vi "suhas&claire-mainencoder.vi"() -> ()   [LabVIEW 2026]
uses:
  <vilib>/DAQmx/read.llb/DAQmx Read (Counter DBL 1Chan 1Samp).vi
  <vilib>/Utility/file.llb/Write Delimited Spreadsheet (string).vi
  <vilib>/DAQmx/miscellaneous.llb/DAQmx Fill In Error Info.vi
panel:
  out "Invert X":bool
  in  "Motor Clock Num per Pulse":u32=100
  in  "Port0 Bits 2":tag="Dev1/port0/line0:7"
  in  "Laser Sync Source":tag="/Dev1/PFI8"
  in  "Laser DO Rate":u32=40000
  in  "Motor Pulse Rate 2":i32=200
  in  "kx":dbl=1.0
  in  "Move X 2":bool
  in  "delta_x 2":dbl=1.0
  in  "xdir 2":bool=TRUE
  out "Y Velocity (mm/s)":dbl
  out "Y Position (mm)":dbl
  out "Time Between Pulse":dbl
  in  "stop":bool
  out "Logging":bool
  out "Saving to":path
  out "XY Graph":cluster{i16[], dbl[]}(graph)
  out "Pulse Count":dbl
  out "X Velocity (mm/s)":dbl
  out "X Position (mm)":dbl
  # "mm"
  # "mm/s"
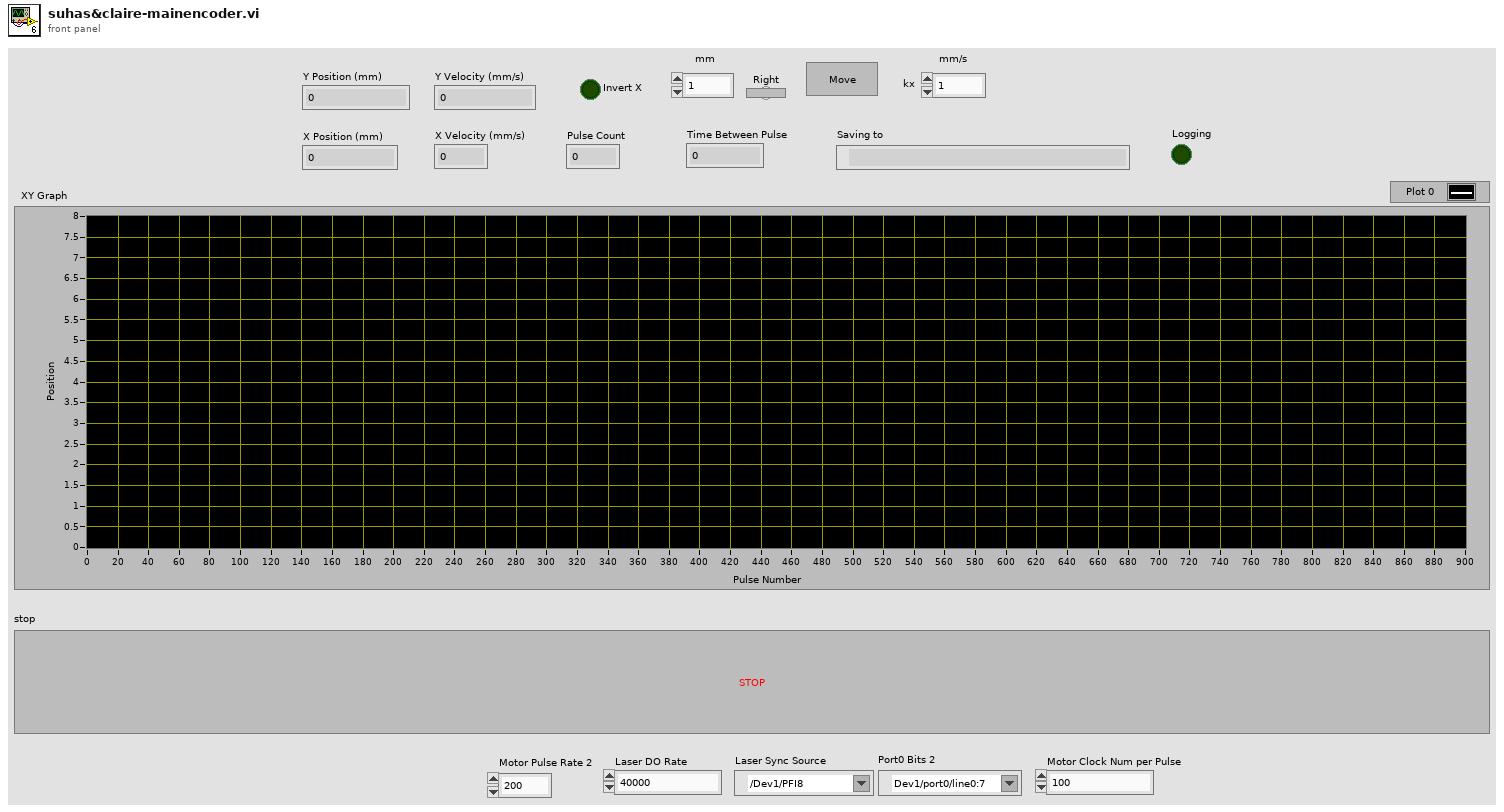
[diagram p1: front panel]
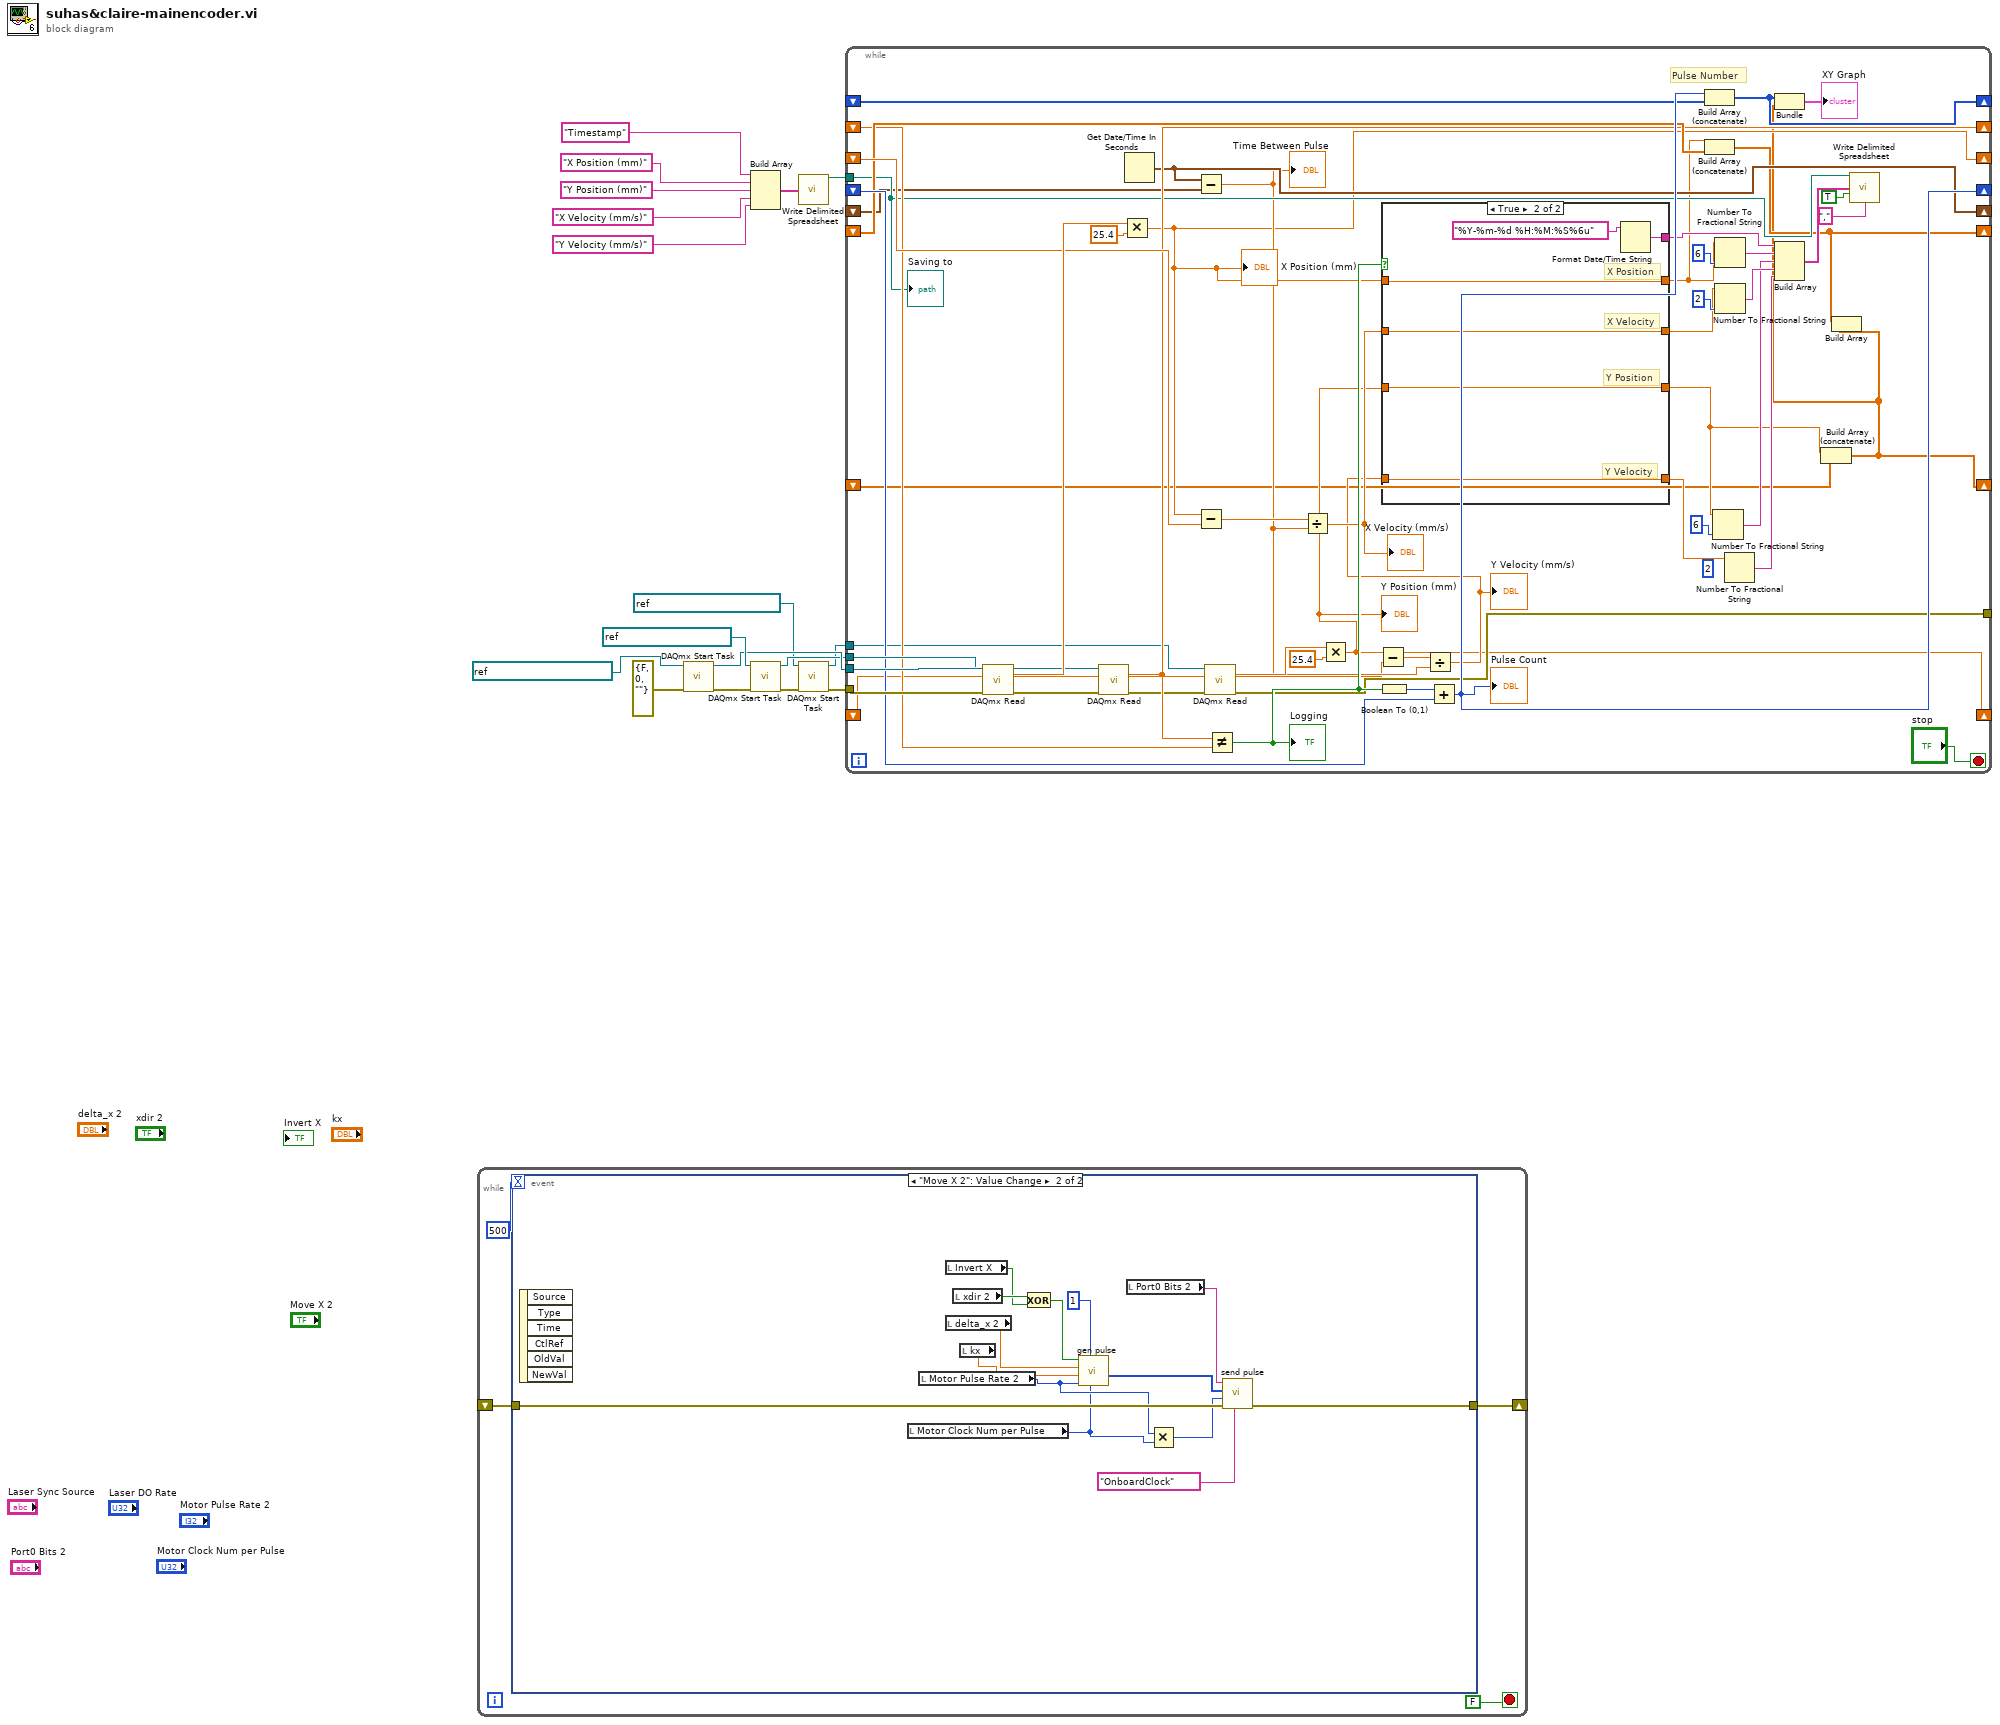
[diagram p0: block diagram]
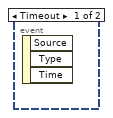
[diagram p2: hidden frame]
diagram:
  n1 = while {
    shift-right: [w20] -> _
    shift-left: _ -> [w19]
    stop <- FALSE stop-if-true
    n2 = event shown="[1] \"Move X 2\": Value Change" {
      selector: _ -> [_ _]
      dyn-events: _ -> [_ _]
      timeout: 500 -> [_ _]
      tunnel: [_ w35] -> w20
      tunnel: w19 -> [_ w34]
      event Timeout {
        n3 = event-data() -> ()  [unwired: 1 in, 3 out]
      }
      event "Move X 2": Value Change {
        n4 = event-data() -> ()  [unwired: 1 in, 6 out]
        n5 = local read "Motor Clock Num per Pulse"() -> (w27:u32)
        n6 = local read "Motor Pulse Rate 2"() -> (w28:i32)
        n7 = local read "Invert X"() -> (w22:bool)
        n8 = local read "delta_x 2"() -> (w32:dbl)
        n9 = local read "xdir 2"() -> (w24:bool)
        n10 = local read "kx"() -> (w31:dbl)
        n11 = Exclusive Or(1:w22, 2:w24) -> (0:w23:bool)
        n12 = call "gen pulse.vi"("clk per pulse"=w27, "bit"=u8 1, "Motor Pulse Rate / mm"=w28, "kx"=w31, "xn"=w32, "dir"=w23) -> ("pulsetrain"=w30:u8[])  [unwired: 3 in, 2 out]
        n13 = local read "Port0 Bits 2"() -> (w29:tag)
        n14 = Multiply(x=w28, y=w27) -> (x*y=w26:u32)
        n15 = call "send pulse.vi"("source"=tag "OnboardClock", "error in"=w34, "Motors DO rate"=w26, "P0 DO data"=w30, "Port0 Bits"=w29) -> ("error out"=w35:errorcluster)  [unwired: 6 in]
      }
    }
  }
  n16 = call <vilib>:"DAQmx Start Task.vi"("task/channels in"=refnum<k21> "MyLinearPositionTask", "error in"=errorcluster {"status"=FALSE, "code"=0, "source"=""}) -> ("task out"=w14:refnum<k21>, "error out"=w8:errorcluster)  [unwired: 12 in]
  n17 = Build Array("Timestamp", "X Position (mm)", "Y Position (mm)", "X Velocity (mm/s)", "Y Velocity (mm/s)") -> (w10:string[])
  n18 = call <vilib>:"DAQmx Start Task.vi"("task/channels in"=refnum<k21> "MyCountEdgesTask", "error in"=w8) -> ("task out"=w13:refnum<k21>, "error out"=w3:errorcluster)  [unwired: 12 in]
  n19 = call-poly <vilib>:"Write Delimited Spreadsheet.vi"("1D data"=w10) -> ("new file path (Not A Path if cancelled)"=w9:path)  [unwired: 13 in, 1 out]
  n20 = call <vilib>:"DAQmx Start Task.vi"("task/channels in"=refnum<k21> "MyLinearPositionTaskY", "error in"=w3) -> ("task out"=w1:refnum<k21>, "error out"=w2:errorcluster)  [unwired: 12 in]
  n21 = while {
    tunnel: w2 -> [w86]
    tunnel: w14 -> [w85]
    tunnel: w13 -> [w82]
    shift-right: [w72] -> _
    shift-left: _ -> [w71]
    shift-right: [w48] -> _
    shift-left: _ -> [w80]
    shift-right: [w76] -> _
    shift-left: _ -> [w77]
    shift-right: [w70] -> _
    shift-left: _ -> [w75]
    shift-right: [w37] -> _
    shift-left: _ -> [w74]
    tunnel: w9 -> [w62]
    shift-right: [w61] -> _
    shift-left: _ -> [w60]
    tunnel: w1 -> [w59]
    tunnel: [w57] -> _
    shift-right: [w43] -> _
    shift-left: _ -> [w42]
    shift-right: [w36] -> _
    shift-left: _ -> [w38]
    stop <- "stop" stop-if-true
    (unwired) i16 2 ("precision (6)")
    # "Pulse Number"
    n22 = call-poly <vilib>:"DAQmx Read.vi"("task/channels in"=w85, "error in"=w86) -> ("data"=w84:dbl, "error out"=w81:errorcluster)  [unwired: 11 in, 1 out]
    n23 = call-poly <vilib>:"DAQmx Read.vi"("task/channels in"=w82, "error in"=w81) -> ("data"=w72:dbl, "error out"=w58:errorcluster)  [unwired: 11 in, 1 out]
    n24 = Multiply(x=w84, y=25.4) -> (x*y=w48:dbl)
    "X Position (mm)" <- w48
    n25 = Get Date/Time In Seconds() -> (seconds since 1Jan1904=w61:timestamp)
    n26 = Subtract(x=w61, y=w60) -> (x-y=w53:dbl)
    "Time Between Pulse" <- w53
    n27 = Subtract(x=w48, y=w80) -> (x-y=w79:dbl)
    n28 = call-poly <vilib>:"DAQmx Read.vi"("task/channels in"=w59, "error in"=w58) -> ("data"=w56:dbl, "error out"=w57:errorcluster)  [unwired: 11 in, 1 out]
    n29 = Not Equal?(x=w72, y=w71) -> (x != y?=w73:bool)
    "Logging" <- w73
    n30 = Divide(x=w79, y=w53) -> (x/y=w47:dbl)
    "X Velocity (mm/s)" <- w47
    n31 = Multiply(x=w56, y=25.4) -> (x*y=w43:dbl)
    "Y Position (mm)" <- w43
    n32 = Subtract(x=w43, y=w42) -> (x-y=w54:dbl)
    n33 = Boolean To (0,1)(Boolean=w73) -> (0, 1=w78:i16)
    n34 = Divide(x=w54, y=w53) -> (x/y=w45:dbl)
    "Y Velocity (mm/s)" <- w45
    n35 = case shown="True" w73 {
      tunnel: [_ w92] -> w67
      tunnel: w48 -> [_ w91]
      tunnel: [_ w91] -> w41
      tunnel: w47 -> [_ w90]
      tunnel: [_ w90] -> w46
      tunnel: w43 -> [_ w89]
      tunnel: [_ w89] -> w39
      tunnel: w45 -> [_ w88]
      tunnel: [_ w88] -> w44
      frame False {
      }
      frame True {
        # "Y Velocity"
        # "Y Position"
        # "X Velocity"
        # "X Position"
        n36 = Format Date/Time String(time format string (%c)="%Y-%m-%d %H:%M:%S%6u") -> (date/time string=w92:string)  [unwired: 2 in]
      }
    }
    n37 = Add(x=w78, y=w77) -> (x+y=w76:i16)
    "Pulse Count" <- w76
    n38 = Build Array (concatenate)(w76, w75) -> (w70:i16[])
    n39 = Build Array (concatenate)(w41, w74) -> (w37:dbl[])
    n40 = Number To Fractional String(number=w39, precision (6)=i16 6) -> (F-format string=w50:string)  [unwired: 2 in]
    n41 = Number To Fractional String(number=w41, precision (6)=i16 6) -> (F-format string=w66:string)  [unwired: 2 in]
    n42 = Number To Fractional String(number=w46, precision (6)=i16 2) -> (F-format string=w52:string)  [unwired: 2 in]
    n43 = Number To Fractional String(number=w44) -> (F-format string=w49:string)  [unwired: 3 in]
    n44 = Build Array(w67, w66, w50, w52, w49) -> (w65:string[])
    n45 = Build Array (concatenate)(w39, w38) -> (w36:dbl[])
    n46 = Bundle(w70, w36) -> (→"XY Graph":cluster{i16[], dbl[]})  [unwired: 1 in]
    n47 = Build Array(w37, w36) -> ()  [unwired: 1 out]
    n48 = call-poly <vilib>:"Write Delimited Spreadsheet.vi"("file path (dialog if empty)"=w62, "1D data"=w65, "append to file? (new file:F)"=TRUE, "delimiter (\\t)"="," ("delimiter (\\t)")) -> ()  [unwired: 10 in, 2 out]
    "Saving to" <- w62
  }
